vi "DF001 - StringToConvertedString.vi"(11 "String (Input)":string) -> (3 "Converted String (Output)":string)   [LabVIEW 2015]
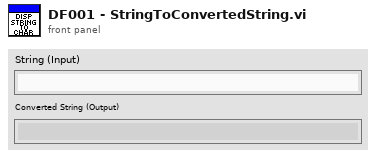
[diagram p1: front panel]
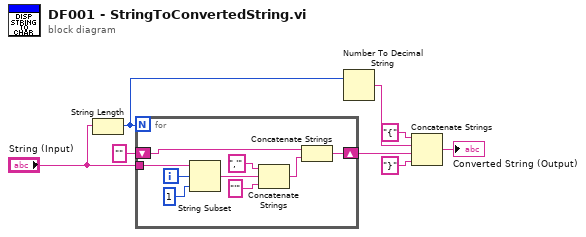
[diagram p0: block diagram]
diagram:
  n1 = String Length(string="String (Input)") -> (length=w5:i32)
  n2 = for {
    N: w5 -> [_]
    tunnel: "String (Input)" -> [w17]
    shift-right: [w10] -> w7
    shift-left: "" -> [w9]
    i -> [w16]
    n3 = String Subset(string=w17, offset (0)=w16, length (rest)=1 ("length (rest)")) -> (substring=w12:string)
    n4 = Concatenate Strings(",'" ("string"), w12, "'" ("string")) -> (w11:string)
    n5 = Concatenate Strings(w9, w11) -> (w10:string)
  }
  n6 = Number To Decimal String(number=w5) -> (decimal integer string=w4:string)  [unwired: 1 in]
  n7 = Concatenate Strings("{" ("string"), w4, w7, "}" ("string")) -> (→"Converted String (Output)":string)
